vi "Write Time (ms).vi"(8 "error in (no error)":errorcluster, 10 "Time (ms)":u32, 11 "bt_Wait in":refnum<class "bt_Wait.lvclass">) -> (0 "error out":errorcluster, 3 "bt_Wait out":refnum<class "bt_Wait.lvclass">)   [LabVIEW 2021, in "BT.lvlib" / "bt_Wait.lvclass"]
uses:
  bt_Wait.lvclass
  bt_Wait.lvclass/bt_Wait.ctl
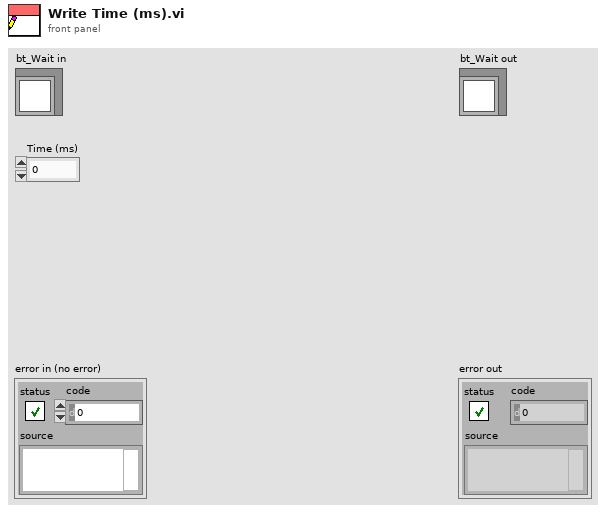
[diagram p1: front panel]
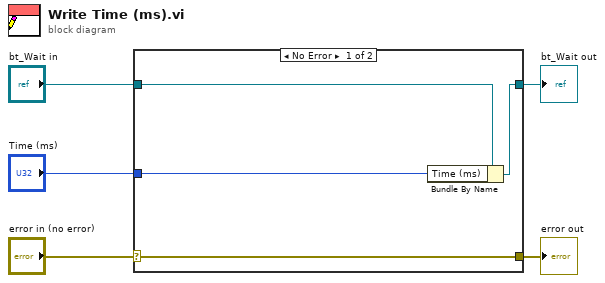
[diagram p0: block diagram]
diagram:
  n1 = case shown="No Error" "error in (no error)" {
    selector: "error in (no error)" -> [w9 w10]
    tunnel: [w9 w10] -> w4
    tunnel: [w7 w11] -> w2
    tunnel: "bt_Wait in" -> [w8 w11]
    tunnel: "Time (ms)" -> [w6 _]
    frame No Error {
      n2 = Bundle By Name(cluster=w8, "Time (ms)"=w6) -> (w7:refnum<class "bt_Wait.lvclass">)
    }
    frame Error {
    }
  }
  "error out" <- w4
  "bt_Wait out" <- w2
